vi "Supervisor_Handle_Event.vi"(8 "error in (no error)":errorcluster={"status"=FALSE, "code"=0, "source"="\"\""}, 10 "RuntimeMessage":string, 11 "Current run state":string) -> (0 "error out":errorcluster={"status"=FALSE, "code"=0, "source"="\"\""}, 2 "status ok":bool, 3 "Updated state and effects":string)   [LabVIEW 2026]
doc: "INTENT: Apply legal state transitions. LOGIC: Enforce Idle Validating Ready Running and stop/fault/shutdown path; reject illegal transitions."
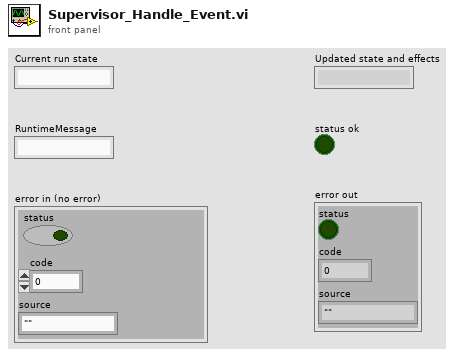
[diagram p1: front panel]
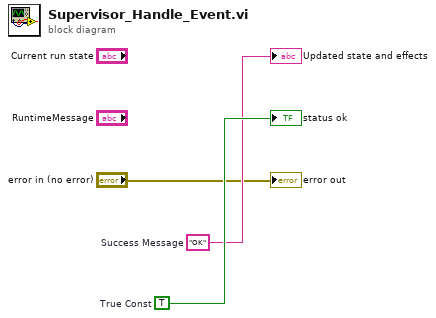
[diagram p0: block diagram]
diagram:
  w3 = TRUE  # True Const
  w2 = "OK"  # Success Message
  "Updated state and effects" <- w2
  "status ok" <- w3
  "error out" <- "error in (no error)"
